vi "Run Tests CLI.vi"(11 "Command Line Arguments":string[](array[string])) -> (2 "Output":string, 3 "Exit Code":i32)   [LabVIEW 2026]
doc: "Headless Caraya runner for CI. Runs every ATM unit test VI in this folder through Caraya's Run Tests.vi with Interactive FALSE (no dialog) and writes a JUnit XML report to results\\caraya-report.xml next to this VI. The results folder is created when missing and an old report is deleted first, so the report is always from this run.\n\nConnector pane follows LabVIEW CLI's RunVI contract - do not change it:\n Command Line Arguments (input, unused)\n Exit Code: 0 when every test passed, 1 when any test failed, Caraya returned an error, or no report was written\n Output: one-line verdict, Caraya's error code and the report path\n\nUsage:\n LabVIEWCLI -OperationName RunVI -VIPath <this VI> -LabVIEWPath <LabVIEW.exe> -PortNumber 3364\n\nThe test VIs are found relative to this VI, so the folder can be checked out anywhere."
uses:
  <vilib>/addons/_JKI Toolkits/Caraya/Caraya.lvlib
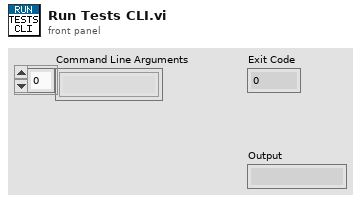
[diagram p1: front panel]
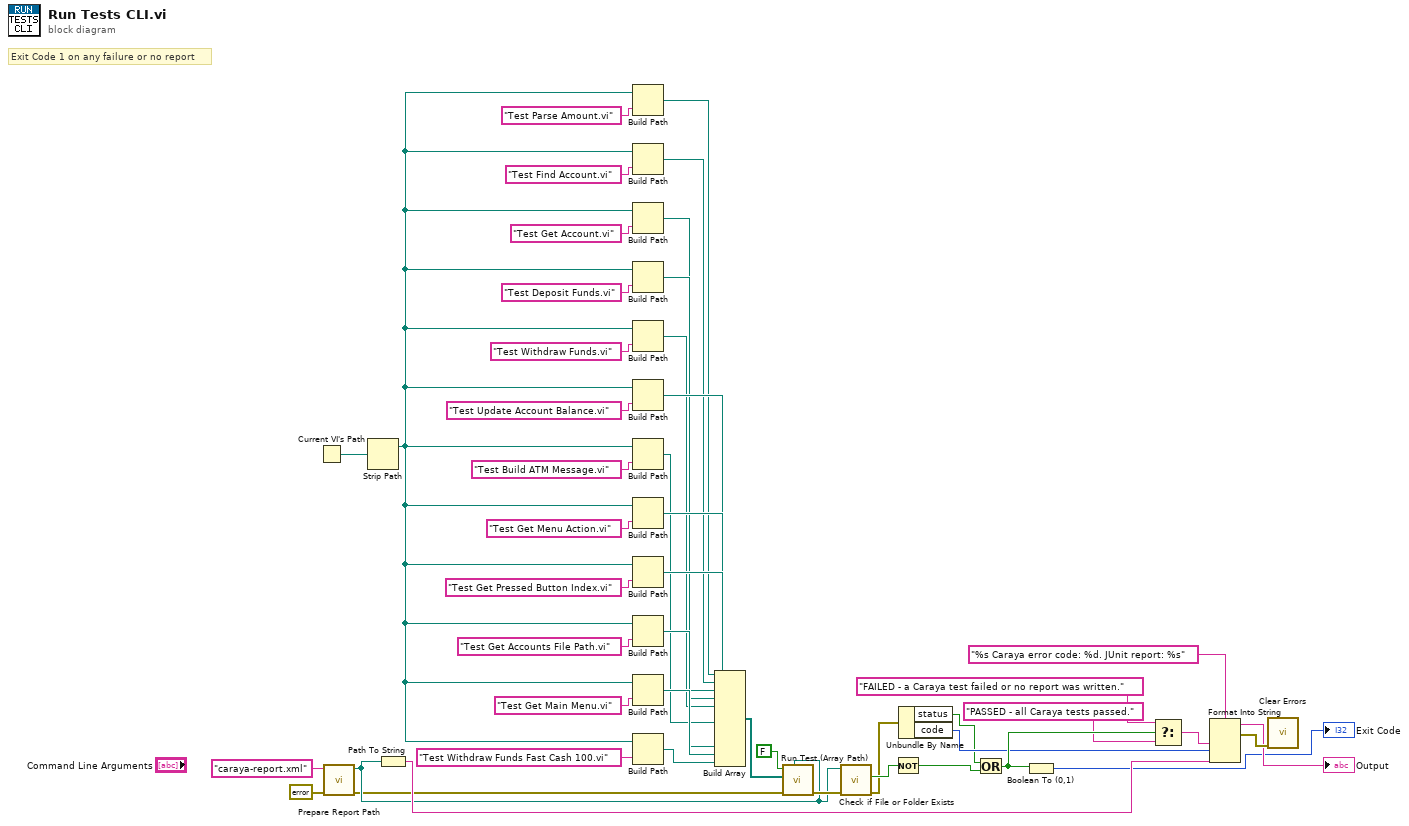
[diagram p0: block diagram]
diagram:
  # "Exit Code 1 on any failure or no report"
  n1 = Current VI's Path() -> (path=w21:path)
  n2 = call "Prepare Report Path.vi"("error in"=errorcluster {"status"=FALSE, "code"=0, "source"=""} ("no error"), "Report File Name"="caraya-report.xml" ("report file name")) -> ("error out"=w22:errorcluster, "Report Path"=w23:path)  [unwired: 8 in]
  n3 = Strip Path(path=w21) -> (stripped path=w24:path)  [unwired: 1 out]
  n4 = Path To String(path=w23) -> (string=w25:string)
  n5 = Build Path(base path=w24, name or relative path="Test Parse Amount.vi" ("name or relative path 1")) -> (appended path=w26:path)
  n6 = Build Path(base path=w24, name or relative path="Test Find Account.vi" ("name or relative path 2")) -> (appended path=w27:path)
  n7 = Build Path(base path=w24, name or relative path="Test Get Account.vi" ("name or relative path 3")) -> (appended path=w28:path)
  n8 = Build Path(base path=w24, name or relative path="Test Deposit Funds.vi" ("name or relative path 4")) -> (appended path=w29:path)
  n9 = Build Path(base path=w24, name or relative path="Test Withdraw Funds.vi" ("name or relative path 5")) -> (appended path=w30:path)
  n10 = Build Path(base path=w24, name or relative path="Test Update Account Balance.vi" ("name or relative path 6")) -> (appended path=w31:path)
  n11 = Build Path(base path=w24, name or relative path="Test Build ATM Message.vi" ("name or relative path 7")) -> (appended path=w32:path)
  n12 = Build Path(base path=w24, name or relative path="Test Get Menu Action.vi" ("name or relative path 8")) -> (appended path=w33:path)
  n13 = Build Path(base path=w24, name or relative path="Test Get Pressed Button Index.vi" ("name or relative path 9")) -> (appended path=w34:path)
  n14 = Build Path(base path=w24, name or relative path="Test Get Accounts File Path.vi" ("name or relative path 10")) -> (appended path=w35:path)
  n15 = Build Path(base path=w24, name or relative path="Test Get Main Menu.vi" ("name or relative path 11")) -> (appended path=w36:path)
  n16 = Build Path(base path=w24, name or relative path="Test Withdraw Funds Fast Cash 100.vi" ("name or relative path 12")) -> (appended path=w37:path)
  n17 = Build Array(w26, w27, w28, w29, w30, w31, w32, w33, w34, w35, w36, w37) -> (w38:path[])
  n18 = call <vilib>:"Run Test (Array Path).vi"("Report Path"=w23, "error in"=w22, "Paths"=w38, "Interactive (T)"=FALSE) -> ("error out"=w39:errorcluster)  [unwired: 6 in, 1 out]
  n19 = call <vilib>:"Check if File or Folder Exists.vi"("error in (no error)"=w39, "path"=w23) -> ("error out"=w40:errorcluster, "file or folder exists?"=w41:bool)  [unwired: 7 in, 1 out]
  n20 = Not(x=w41) -> (.not. x?=w44:bool)
  n21 = Unbundle By Name(w40) -> ("status"=w42:bool, "code"=w43:i32)
  n22 = Or(x=w42, y=w44) -> (x .or. y?=w45:bool)
  n23 = Boolean To (0,1)(Boolean=w45) -> (0, 1=→"Exit Code":i16)
  n24 = Select(t="FAILED - a Caraya test failed or no report was written." ("Failed Verdict"), s=w45, f="PASSED - all Caraya tests passed." ("Passed Verdict")) -> (s? t:f=w46:string)
  n25 = Format Into String(format string="%s Caraya error code: %d. JUnit report: %s" ("Output Format"), w46, w43, w25) -> (resulting string=→"Output":string, error out=w47:errorcluster)  [unwired: 2 in]
  n26 = call <vilib>:"Clear Errors.vi"("error in (no error)"=w47) -> ()  [unwired: 5 in, 2 out]
